vi "Do Save VI.vi"(8 "error in (no error)":errorcluster, 10 "save_vi Argument":T3, 11 "Data Cluster in":T1) -> (0 "error out":errorcluster, 2 "VI Path":path, 3 "Data Cluster out":T1)   [LabVIEW 2020, in "Scripting Server.lvlib"]
uses:
  Scripting Server.lvlib
  Module Data--cluster.ctl
  Config Data.ctl
  save_vi Argument--cluster.ctl
  save_vi (Reply Payload)--cluster.ctl
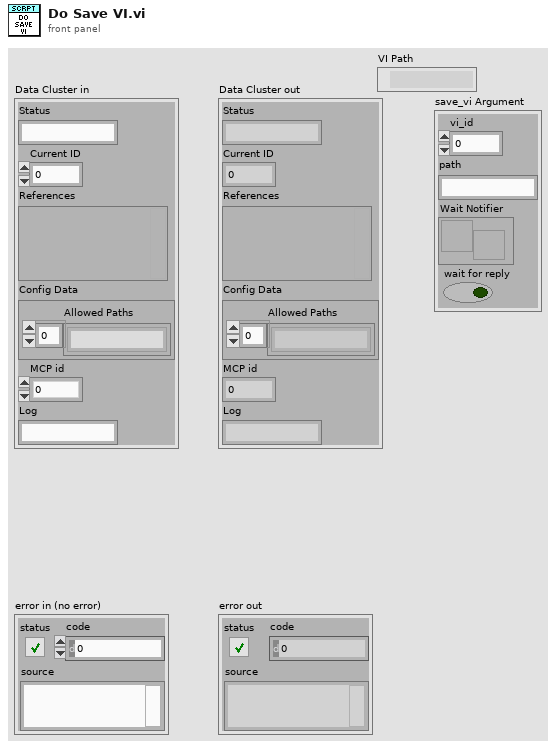
[diagram p1: front panel]
types:
  T1 = typedef "Scripting Server.lvlib/Module Data--cluster.ctl" = cluster{"Status":string, "Current ID":i32, "References":variant, "Config Data":T2, "MCP id":i32, "Log":string}
  T2 = typedef "Scripting Server.lvlib/Config Data.ctl" = cluster{"Allowed Paths":string[]}
  T3 = typedef "Scripting Server.lvlib/save_vi Argument--cluster.ctl" = cluster{"vi_id":i32, "path":string, "Wait Notifier":refnum<notifier>, "wait for reply":bool}
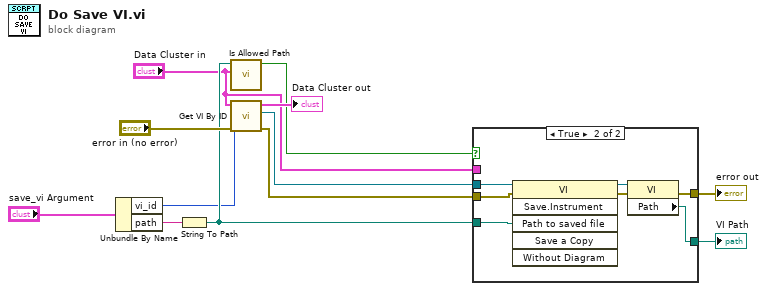
[diagram p0: block diagram]
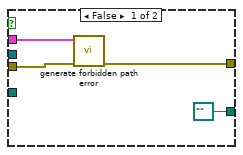
[diagram p2: hidden frame]
diagram:
  n1 = Unbundle By Name("save_vi Argument") -> ("vi_id"=w1:i32, "path"=w7:string)
  n2 = String To Path(string=w7) -> (path=w4:path)
  n3 = call "Is Allowed Path.vi"("Data Cluster in"="Data Cluster in", "Path"=w4) -> ("Forbidden"=w3:bool)  [unwired: 9 in]
  n4 = call "Get VI By ID.vi"("error in (no error)"="error in (no error)", "ID"=w1, "Data Cluster in"="Data Cluster in") -> ("error out"=w10:errorcluster, "VI Reference"=w8:refnum<vi>, "Data Cluster out"=→"Data Cluster out":T1)  [unwired: 6 in]
  n5 = case shown="True" w3 {
    tunnel: w10 -> [w16 w23]
    tunnel: w8 -> [_ w21]
    tunnel: [w14 w20] -> w6
    tunnel: [path "" ("Path") w18] -> w5
    tunnel: w4 -> [_ w17]
    tunnel: "Data Cluster in" -> [w13 _]
    frame False {
      n6 = call "generate forbidden path error.vi"("error in (no error)"=w16, "Data Cluster in"=w13) -> ("error out"=w14:errorcluster)  [unwired: 9 in]
    }
    frame True {
      n7 = invoke on="Invoke Node" class="VI" method="Save.Instrument"(reference=w21, error in=w23, "Path to saved file"=w17) -> (reference out=w19:refnum<vi>, error out=w22:errorcluster)  [unwired: 3 in, 4 out]
      n8 = property on="Property Node" class="VI"(reference=w19, error in=w22) -> (error out=w20:errorcluster, "Path"=w18:path)  [unwired: 1 out]
    }
  }
  "error out" <- w6
  "VI Path" <- w5
